vi "Create Notch Filter (FGV).vi"(6 "fs (Hz)":dbl, 7 "init [F]":bool, 8 "error in (no error)":errorcluster) -> (0 "error out":errorcluster, 2 "IIR Filters":T1(array[cluster]), 5 "init?":bool)   [LabVIEW 2019, in "DSP.lvclass"]
uses:
  DSP.lvclass
panel:
  out "concatenated string":string
  out "harmonics":i32
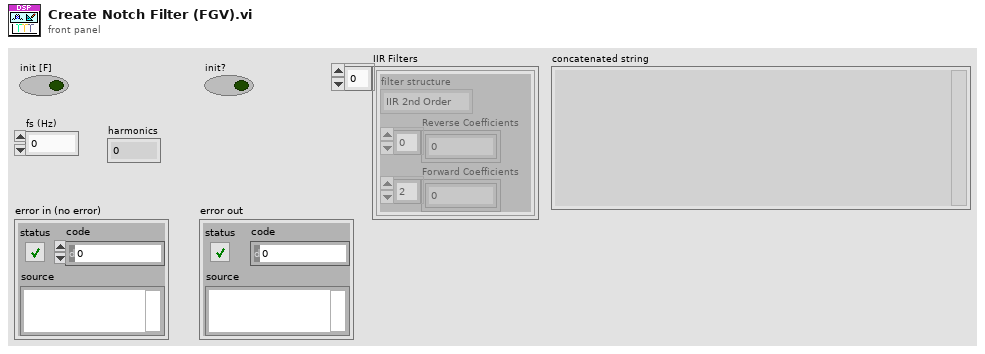
[diagram p1: front panel]
types:
  T1 = cluster{"filter structure":enum32{"IIR 2nd Order", "IIR 4th Order"}, "Reverse Coefficients":dbl[], "Forward Coefficients":dbl[]}[]
  T2 = cluster{"filter structure":enum32{"IIR 2nd Order", "IIR 4th Order"}, "Reverse Coefficients":dbl[], "Forward Coefficients":dbl[]}
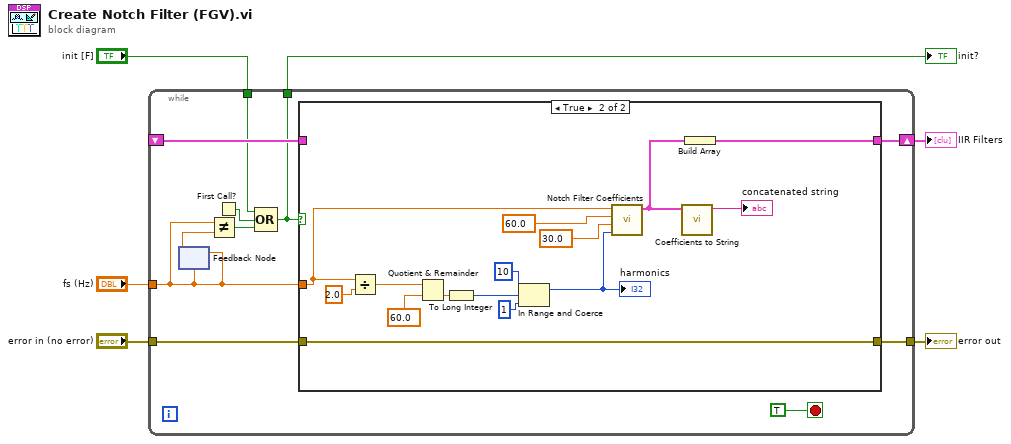
[diagram p0: block diagram]
diagram:
  n1 = while {
    shift-right: [w16] -> w1
    shift-left: _ -> [w9]
    tunnel: "fs (Hz)" -> [w15]
    tunnel: "error in (no error)" -> [w17]
    tunnel: [w10] -> w4
    tunnel: "init [F]" -> [w8]
    tunnel: [w7] -> w6
    stop <- TRUE stop-if-true
    n2 = feedback #1(w15) -> (w14:dbl)
    n3 = feedback-in #1(w15) -> ()
    n4 = Not Equal?(x=w15, y=w14) -> (x != y?=w13:bool)
    n5 = First Call?() -> (First Call?: T/F=w12:bool)
    n6 = Compound Arithmetic op=OR(w8, w12, w13) -> (w7:bool)
    n7 = case shown="True" w7 {
      tunnel: w17 -> [w18 w34]
      tunnel: [w19 w29] -> w16
      tunnel: w15 -> [_ w20]
      tunnel: [w18 w34] -> w10
      tunnel: w9 -> [w19 _]
      frame False {
      }
      frame True {
        n8 = Divide(x=w20, y=2.0) -> (x/y=w23:dbl)
        n9 = Quotient & Remainder(x=w23, y=60.0 ("f0 [Hz]")) -> (floor(x/y)=w33:dbl)  [unwired: 1 out]
        n10 = To Long Integer(number=w33) -> (32bit integer=w22:i32)
        n11 = In Range and Coerce(upper limit=10, x=w22, lower limit=1) -> (coerced(x)=w26:i32)  [unwired: 1 out]
        "harmonics" <- w26
        n12 = call "Notch Filter Coefficients.vi"("harmonics"=w26, "Q"=30.0 ("Q factor"), "notch (Hz)"=60.0 ("Q factor"), "Sample rate (Hz)"=w20) -> ("IIR Filter Cluster"=w21:T2)  [unwired: 5 in, 2 out]
        n13 = call "Coefficients to String.vi"("IIR Filter Cluster"=w21) -> ("String"=→"concatenated string":string)  [unwired: 10 in]
        n14 = Build Array(w21) -> (w29:T1)
      }
    }
  }
  "init?" <- w6
  "IIR Filters" <- w1
  "error out" <- w4
